vi "White--constant.vi"() -> (1 "White":u32(colorbox))   [LabVIEW 2018, in "Band Colors.lvlib"]
doc: "Provides the RGB color value for white.\n\nThe VI converts the RGB components (255, 255, 255) into a LabVIEW color value and returns it through <b>White</b>."
uses:
  Band Colors.lvlib
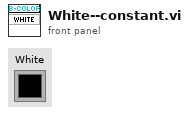
[diagram p1: front panel]
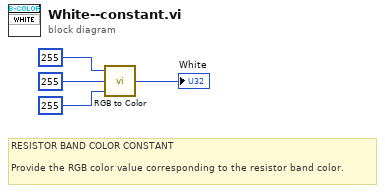
[diagram p0: block diagram]
diagram:
  # "RESISTOR BAND COLOR CONSTANT\n\nProvide the RGB color value corresponding to the resistor band color."
  n1 = call <vilib>:"RGB to Color.vi"("B"=u8 255, "G"=u8 255, "R"=u8 255) -> ("Color"=→"White":u32)
